vi "Energy_Meter_Control.vi"(7 "error in":T3, 8 "State":T2) -> (0 "error out":errorcluster, 3 "Resource out":refnum<visa-resource-name>)   [LabVIEW 2021]
uses:
  Support/Relay_no.ctl
  State.ctl
  <vilib>/NI/Modbus Library/API/Wrapper/Create Serial Master.vi
  <vilib>/NI/Modbus Library/API/Master/Modbus Master.lvclass
  <vilib>/NI/Modbus Library/API/Wrapper/API Main.lvlib
panel:
  in  "Enum":T1
  out "Frequency":sgl
  out "Apparent Power":sgl
  out "Reactive Power":sgl
  out "Active Power":sgl
  out "Power Factor":sgl
  out "Current":sgl
  out "AC Voltage":sgl
  in  "Resource In":refnum<visa-resource-name>
  # "UART TX"
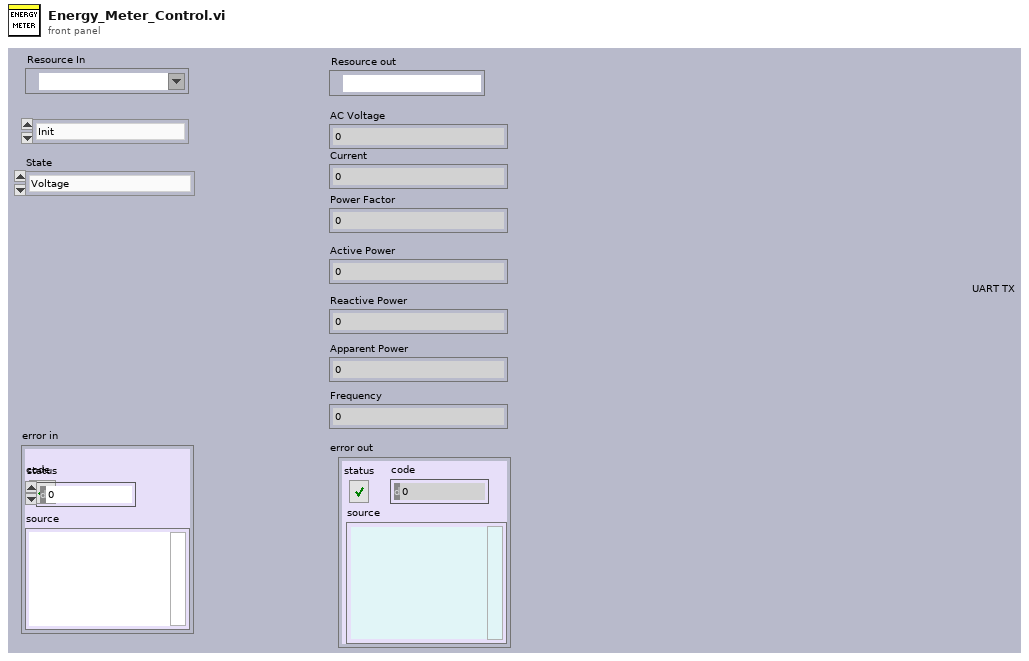
[diagram p1: front panel]
types:
  T1 = typedef "State.ctl" = enum16{"Init", "Close"}
  T2 = typedef "Relay_no.ctl" = enum16{"Voltage", "Current", "Power Factor", "Active Power", "Reactive Power", "Apparent Power", "Frequency"}
  T3 = cluster{"status":bool, "\ncode":i32, "source":string}
  T4 = cluster{"baud rate":u32, "data bits":u16, "parity":enum16{"None", "Odd", "Even", "Mark", "Space"}, "stop bits":u16, "flow control":u16}
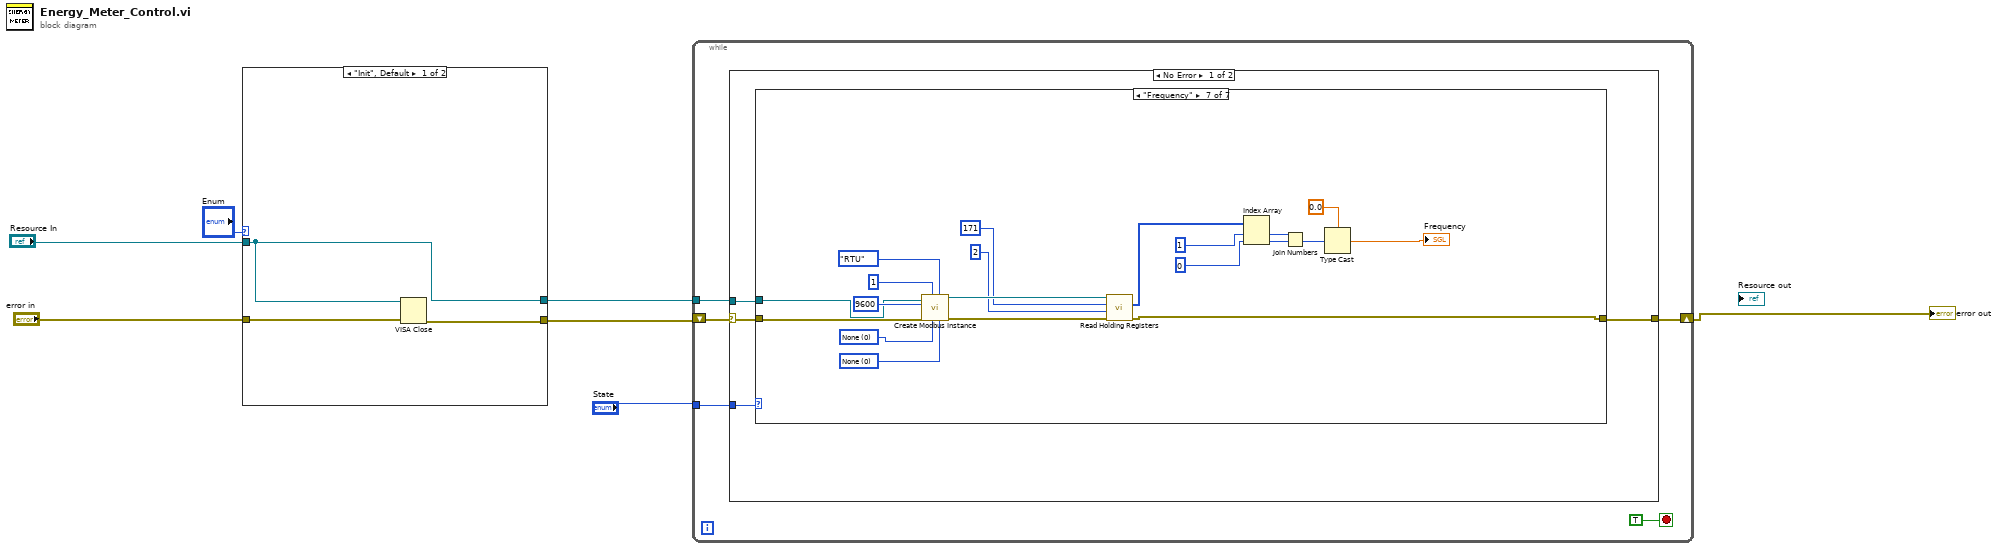
[diagram p0: block diagram]
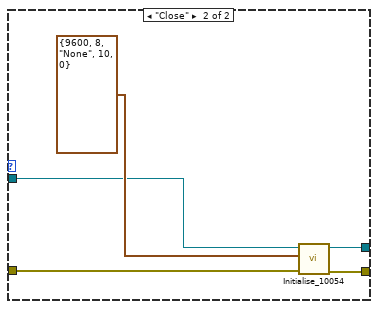
[diagram p2: hidden frame]
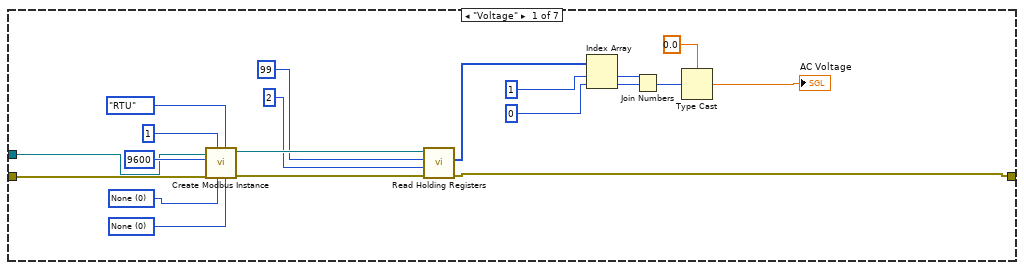
[diagram p3: hidden frame]
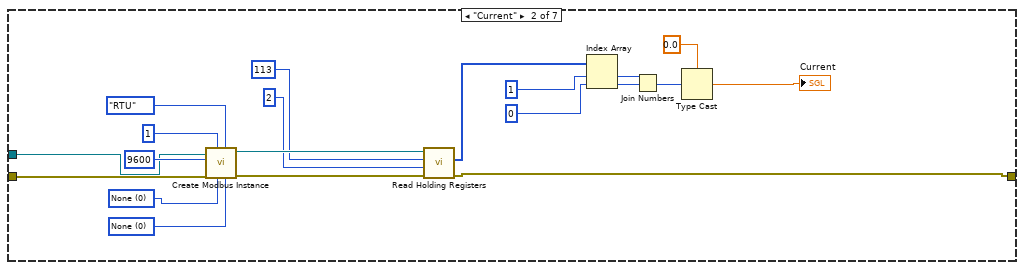
[diagram p4: hidden frame]
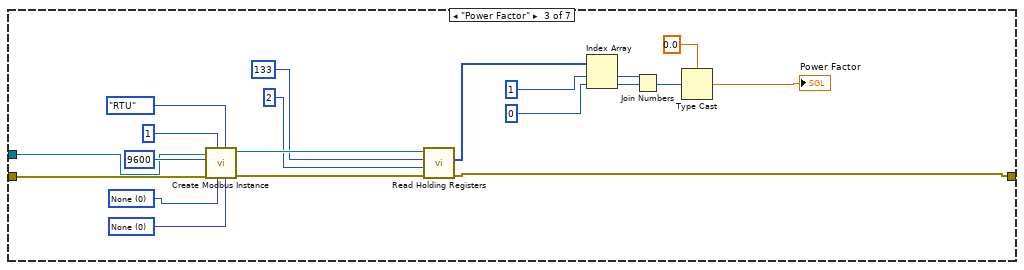
[diagram p5: hidden frame]
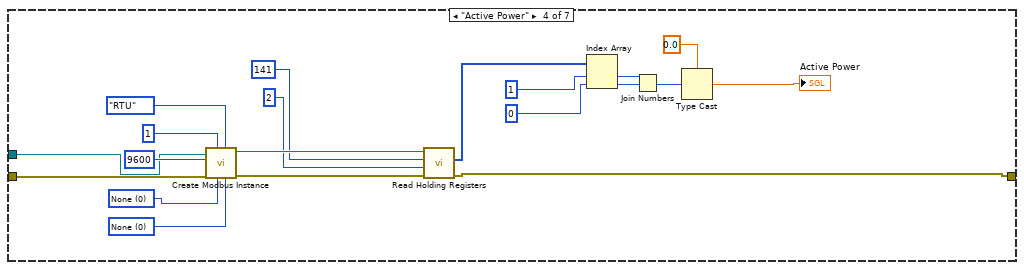
[diagram p6: hidden frame]
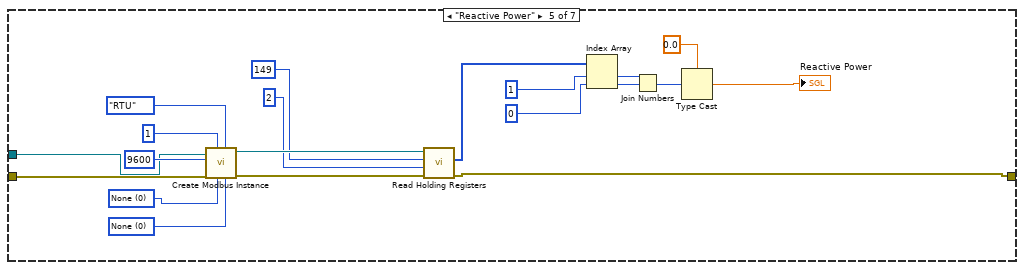
[diagram p7: hidden frame]
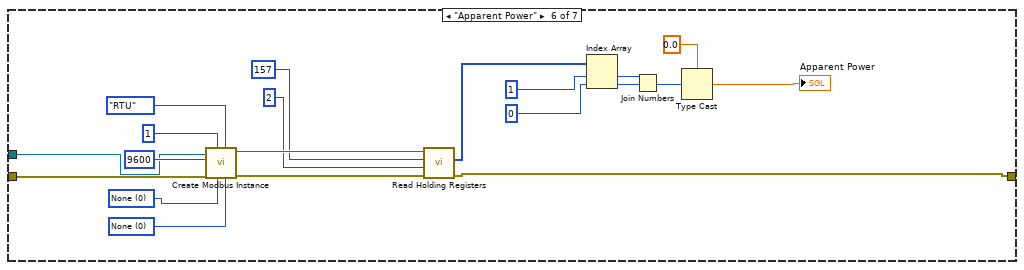
[diagram p8: hidden frame]
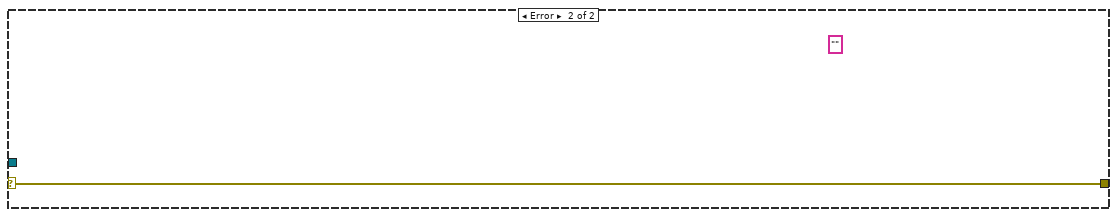
[diagram p9: hidden frame]
diagram:
  n1 = case shown="\"Init\", Default" "Enum" {
    tunnel: "Resource In" -> [w8 w14]
    tunnel: [w8 w13] -> w4
    tunnel: "error in" -> [w10 w12]
    tunnel: [w9 w11] -> w2
    frame "Init", Default {
      n2 = VISA Close(VISA resource name=w8, error in (no error)=w10) -> (error out=w9:errorcluster)
    }
    frame "Close" {
      n3 = call "Initialise_10054 .vi"("error in"=w12, "Serial Settings"=T4 {"baud rate"=9600, "data bits"=8, "parity"=enum."None", "stop bits"=10, "flow control"=0}, "RS232 name in"=w14) -> ("error out"=w11:errorcluster, "RS232 name out"=w13:refnum<visa-resource-name>)  [unwired: 7 in]
    }
  }
  n4 = while {
    tunnel: "State" -> [w19]
    shift-right: [w18] -> w6
    shift-left: w2 -> [w17]
    tunnel: w4 -> [w16]
    stop <- TRUE stop-if-true
    n5 = case shown="No Error" w17 {
      selector: w17 -> [w22 w165]
      tunnel: w19 -> [w24 _]
      tunnel: [w23 w165] -> w18
      tunnel: w16 -> [w21 _]
      frame No Error {
        n6 = case shown="\"Frequency\"" w24 {
          tunnel: w22 -> [w35 w55 w75 w95 w115 w135 w155]
          tunnel: [w25 w45 w65 w85 w105 w125 w145] -> w23
          tunnel: w21 -> [w32 w52 w72 w92 w112 w132 w152]
          frame "Voltage" {
            w44 = u16 0 items=["None", "XON/XOFF", "RTS/CTS", "XON/XOFF & RTS/CTS", "DTR/DSR", "XON/XOFF & DTR/DSR"] ("flow control (none)")
            w40 = u16 0 items=["None", "Odd", "Even", "Mark", "Space"] ("parity (even)")
            n7 = call-poly <vilib>:"Create Modbus Instance.vi"("flow control (none)"=w44, "serial type"=enum16{"RTU", "ASCII"}."RTU", "parity (even)"=w40, "unit ID"=u8 1, "error in"=w35, "baud rate"=u32 9600, "VISA resource name"=w32) -> ("error out"=w39:errorcluster, "serial master instance"=w38:refnum<class "Modbus Master.lvclass">)  [unwired: 3 in]
            n8 = call-dynamic "Read Holding Registers.vi"("error in"=w39, "number of inputs"=u16 2, "starting address"=u16 99, "Modbus master in"=w38) -> ("error out"=w25:errorcluster, "register values"=w34:u16[])  [unwired: 5 in, 1 out]
            n9 = Index Array "Index Array"(array=w34, index #1=1 ("index"), index #2=0 ("index")) -> (element #1=w33:u16, element #2=w30:u16)
            n10 = Join Numbers(hi=w33, lo=w30) -> ((hi.lo)=w29:u32)
            n11 = Type Cast(type=sgl 0.0 ("element"), x=w29) -> (*(type *) &x=→"AC Voltage":sgl)
          }
          frame "Current" {
            w64 = u16 0 items=["None", "XON/XOFF", "RTS/CTS", "XON/XOFF & RTS/CTS", "DTR/DSR", "XON/XOFF & DTR/DSR"] ("flow control (none)")
            w60 = u16 0 items=["None", "Odd", "Even", "Mark", "Space"] ("parity (even)")
            n12 = call-poly <vilib>:"Create Modbus Instance.vi"("flow control (none)"=w64, "serial type"=enum16{"RTU", "ASCII"}."RTU", "parity (even)"=w60, "unit ID"=u8 1, "error in"=w55, "baud rate"=u32 9600, "VISA resource name"=w52) -> ("error out"=w59:errorcluster, "serial master instance"=w58:refnum<class "Modbus Master.lvclass">)  [unwired: 3 in]
            n13 = call-dynamic "Read Holding Registers.vi"("error in"=w59, "number of inputs"=u16 2, "starting address"=u16 113, "Modbus master in"=w58) -> ("error out"=w45:errorcluster, "register values"=w54:u16[])  [unwired: 5 in, 1 out]
            n14 = Index Array "Index Array"(array=w54, index #1=1 ("index"), index #2=0 ("index")) -> (element #1=w53:u16, element #2=w50:u16)
            n15 = Join Numbers(hi=w53, lo=w50) -> ((hi.lo)=w49:u32)
            n16 = Type Cast(type=sgl 0.0 ("element"), x=w49) -> (*(type *) &x=→"Current":sgl)
          }
          frame "Power Factor" {
            w84 = u16 0 items=["None", "XON/XOFF", "RTS/CTS", "XON/XOFF & RTS/CTS", "DTR/DSR", "XON/XOFF & DTR/DSR"] ("flow control (none)")
            w80 = u16 0 items=["None", "Odd", "Even", "Mark", "Space"] ("parity (even)")
            n17 = call-poly <vilib>:"Create Modbus Instance.vi"("flow control (none)"=w84, "serial type"=enum16{"RTU", "ASCII"}."RTU", "parity (even)"=w80, "unit ID"=u8 1, "error in"=w75, "baud rate"=u32 9600, "VISA resource name"=w72) -> ("error out"=w79:errorcluster, "serial master instance"=w78:refnum<class "Modbus Master.lvclass">)  [unwired: 3 in]
            n18 = call-dynamic "Read Holding Registers.vi"("error in"=w79, "number of inputs"=u16 2, "starting address"=u16 133, "Modbus master in"=w78) -> ("error out"=w65:errorcluster, "register values"=w74:u16[])  [unwired: 5 in, 1 out]
            n19 = Index Array "Index Array"(array=w74, index #1=1 ("index"), index #2=0 ("index")) -> (element #1=w73:u16, element #2=w70:u16)
            n20 = Join Numbers(hi=w73, lo=w70) -> ((hi.lo)=w69:u32)
            n21 = Type Cast(type=sgl 0.0 ("element"), x=w69) -> (*(type *) &x=→"Power Factor":sgl)
          }
          frame "Active Power" {
            w104 = u16 0 items=["None", "XON/XOFF", "RTS/CTS", "XON/XOFF & RTS/CTS", "DTR/DSR", "XON/XOFF & DTR/DSR"] ("flow control (none)")
            w100 = u16 0 items=["None", "Odd", "Even", "Mark", "Space"] ("parity (even)")
            n22 = call-poly <vilib>:"Create Modbus Instance.vi"("flow control (none)"=w104, "serial type"=enum16{"RTU", "ASCII"}."RTU", "parity (even)"=w100, "unit ID"=u8 1, "error in"=w95, "baud rate"=u32 9600, "VISA resource name"=w92) -> ("error out"=w99:errorcluster, "serial master instance"=w98:refnum<class "Modbus Master.lvclass">)  [unwired: 3 in]
            n23 = call-dynamic "Read Holding Registers.vi"("error in"=w99, "number of inputs"=u16 2, "starting address"=u16 141, "Modbus master in"=w98) -> ("error out"=w85:errorcluster, "register values"=w94:u16[])  [unwired: 5 in, 1 out]
            n24 = Index Array "Index Array"(array=w94, index #1=1 ("index"), index #2=0 ("index")) -> (element #1=w93:u16, element #2=w90:u16)
            n25 = Join Numbers(hi=w93, lo=w90) -> ((hi.lo)=w89:u32)
            n26 = Type Cast(type=sgl 0.0 ("element"), x=w89) -> (*(type *) &x=→"Active Power":sgl)
          }
          frame "Reactive Power" {
            w124 = u16 0 items=["None", "XON/XOFF", "RTS/CTS", "XON/XOFF & RTS/CTS", "DTR/DSR", "XON/XOFF & DTR/DSR"] ("flow control (none)")
            w120 = u16 0 items=["None", "Odd", "Even", "Mark", "Space"] ("parity (even)")
            n27 = call-poly <vilib>:"Create Modbus Instance.vi"("flow control (none)"=w124, "serial type"=enum16{"RTU", "ASCII"}."RTU", "parity (even)"=w120, "unit ID"=u8 1, "error in"=w115, "baud rate"=u32 9600, "VISA resource name"=w112) -> ("error out"=w119:errorcluster, "serial master instance"=w118:refnum<class "Modbus Master.lvclass">)  [unwired: 3 in]
            n28 = call-dynamic "Read Holding Registers.vi"("error in"=w119, "number of inputs"=u16 2, "starting address"=u16 149, "Modbus master in"=w118) -> ("error out"=w105:errorcluster, "register values"=w114:u16[])  [unwired: 5 in, 1 out]
            n29 = Index Array "Index Array"(array=w114, index #1=1 ("index"), index #2=0 ("index")) -> (element #1=w113:u16, element #2=w110:u16)
            n30 = Join Numbers(hi=w113, lo=w110) -> ((hi.lo)=w109:u32)
            n31 = Type Cast(type=sgl 0.0 ("element"), x=w109) -> (*(type *) &x=→"Reactive Power":sgl)
          }
          frame "Apparent Power" {
            w144 = u16 0 items=["None", "XON/XOFF", "RTS/CTS", "XON/XOFF & RTS/CTS", "DTR/DSR", "XON/XOFF & DTR/DSR"] ("flow control (none)")
            w140 = u16 0 items=["None", "Odd", "Even", "Mark", "Space"] ("parity (even)")
            n32 = call-poly <vilib>:"Create Modbus Instance.vi"("flow control (none)"=w144, "serial type"=enum16{"RTU", "ASCII"}."RTU", "parity (even)"=w140, "unit ID"=u8 1, "error in"=w135, "baud rate"=u32 9600, "VISA resource name"=w132) -> ("error out"=w139:errorcluster, "serial master instance"=w138:refnum<class "Modbus Master.lvclass">)  [unwired: 3 in]
            n33 = call-dynamic "Read Holding Registers.vi"("error in"=w139, "number of inputs"=u16 2, "starting address"=u16 157, "Modbus master in"=w138) -> ("error out"=w125:errorcluster, "register values"=w134:u16[])  [unwired: 5 in, 1 out]
            n34 = Index Array "Index Array"(array=w134, index #1=1 ("index"), index #2=0 ("index")) -> (element #1=w133:u16, element #2=w130:u16)
            n35 = Join Numbers(hi=w133, lo=w130) -> ((hi.lo)=w129:u32)
            n36 = Type Cast(type=sgl 0.0 ("element"), x=w129) -> (*(type *) &x=→"Apparent Power":sgl)
          }
          frame "Frequency" {
            w164 = u16 0 items=["None", "XON/XOFF", "RTS/CTS", "XON/XOFF & RTS/CTS", "DTR/DSR", "XON/XOFF & DTR/DSR"] ("flow control (none)")
            w160 = u16 0 items=["None", "Odd", "Even", "Mark", "Space"] ("parity (even)")
            n37 = call-poly <vilib>:"Create Modbus Instance.vi"("flow control (none)"=w164, "serial type"=enum16{"RTU", "ASCII"}."RTU", "parity (even)"=w160, "unit ID"=u8 1, "error in"=w155, "baud rate"=u32 9600, "VISA resource name"=w152) -> ("error out"=w159:errorcluster, "serial master instance"=w158:refnum<class "Modbus Master.lvclass">)  [unwired: 3 in]
            n38 = call-dynamic "Read Holding Registers.vi"("error in"=w159, "number of inputs"=u16 2, "starting address"=u16 171, "Modbus master in"=w158) -> ("error out"=w145:errorcluster, "register values"=w154:u16[])  [unwired: 5 in, 1 out]
            n39 = Index Array "Index Array"(array=w154, index #1=1 ("index"), index #2=0 ("index")) -> (element #1=w153:u16, element #2=w150:u16)
            n40 = Join Numbers(hi=w153, lo=w150) -> ((hi.lo)=w149:u32)
            n41 = Type Cast(type=sgl 0.0 ("element"), x=w149) -> (*(type *) &x=→"Frequency":sgl)
          }
        }
      }
      frame Error {
        (unwired) "" ("read buffer")
      }
    }
  }
  "error out" <- w6
